vi "~Chart Buffer.vi"(9 "buff size":i32=100, 11 "point":cluster{"x":dbl, "y":dbl} {"y" format="%.2f"; "x" format="%.2f"}) -> (3 "buff out":cluster{"x":dbl, "y":dbl}[](array[cluster]) {"y" format="%.2f"; "x" format="%.2f"})   [LabVIEW 2021]
doc: "::: CalcExpress Toolkit :::\nCopyright (c) 2000-2026 Konstantin Shifershteyn. All rights reserved."
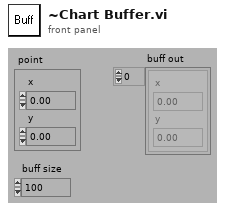
[diagram p1: front panel]
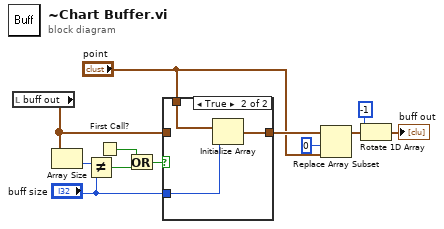
[diagram p0: block diagram]
diagram:
  n1 = local read "buff out"() -> (w4:cluster{"x":dbl, "y":dbl}[])
  n2 = Array Size(array=w4) -> (size(s)=w10:i32)
  n3 = Not Equal?(x=w10, y="buff size") -> (x != y?=w2:bool)
  n4 = First Call?() -> (First Call?: T/F=w1:bool)
  n5 = Or(x=w1, y=w2) -> (x .or. y?=w9:bool)
  n6 = case shown="True" w9 {
    tunnel: [w13 w15] -> w11
    tunnel: w4 -> [w13 _]
    tunnel: "point" -> [_ w14]
    tunnel: "buff size" -> [_ w16]
    frame False {
    }
    frame True {
      n7 = Initialize Array(w14, w16) -> (w15:cluster{"x":dbl, "y":dbl}[])
    }
  }
  n8 = Replace Array Subset(array=w11, new element="point", index=0) -> (w12:cluster{"x":dbl, "y":dbl}[])
  n9 = Rotate 1D Array(1:w12, 2:-1 ("n")) -> (0:→"buff out":cluster{"x":dbl, "y":dbl}[])
